vi "RemoteVI Connect VI Server.vi"(0 "window":u64, 1 "address":string) -> (4 "connected?":bool, 6 "VI":refnum<vi>, 7 "hooks":refnum<vi>, 8 "VI name":string, 9 "mode":string)   [LabVIEW 2020, in "RemoteVI.lvlib"]
doc: "The VI Server route of a window share (docs\\architecture.md, Window targets): when window belongs to ANOTHER LabVIEW process that runs VI Server, opens an application reference to it (Open Application Reference), finds the running VI whose open front panel is window - opened by the window title (a built application answers Application:All VIs In Memory with error 1032, measured), then checked with Front Panel Window:OS Window and Execution:State; a panel with a custom window title is not found and opens RemoteVI Remote Hooks.vi there from the packed library builds\\RemoteVI Hooks\\RemoteVI Hooks.lvlibp (or RemoteVI Hooks.lvlibp next to RemoteVI's folder; a built application can only load compiled code). address: empty = read the application's INI file (<exe>.ini next to the process, server.tcp.enabled=True, server.tcp.port, default 3363) and connect to 127.0.0.1; off = do not try; host:port = that VI Server. connected? TRUE: VI (the shared VI there), hooks and VI name are valid and the share runs with full features (modifier keys, tip strips, splitter bars through the hooks; everything else as for a VI of this LabVIEW). FALSE: window only; mode says why. Called by RemoteVI Server Setup.vi inside the server loop, so the references live as long as the share."
uses:
  RemoteVI.lvlib
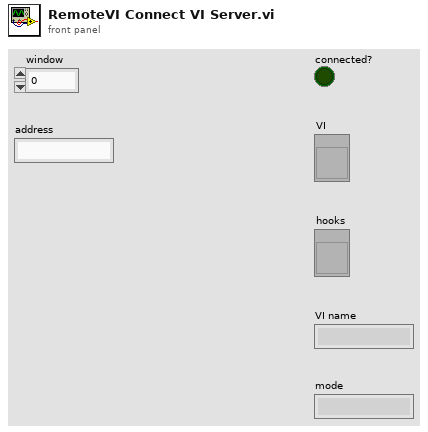
[diagram p1: front panel]
types:
  T1 = enum32{"Bad", "Idle", "Run top level", "Running"}
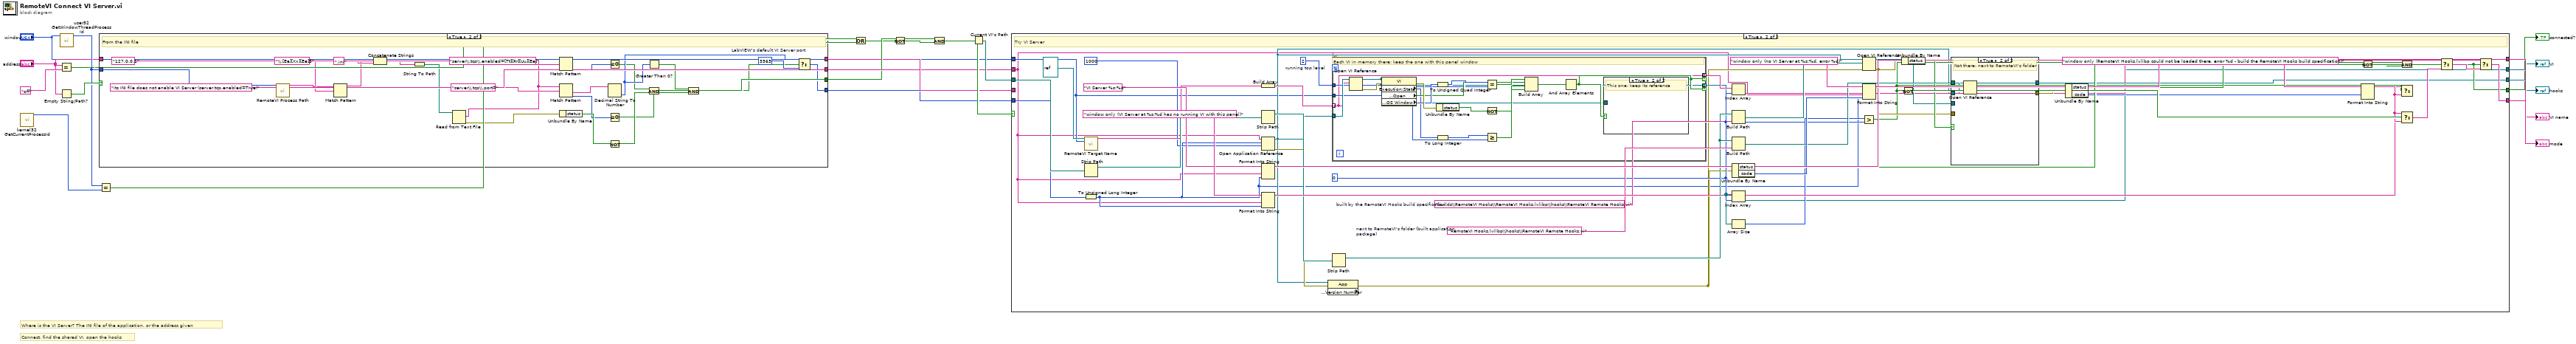
[diagram p0: block diagram]
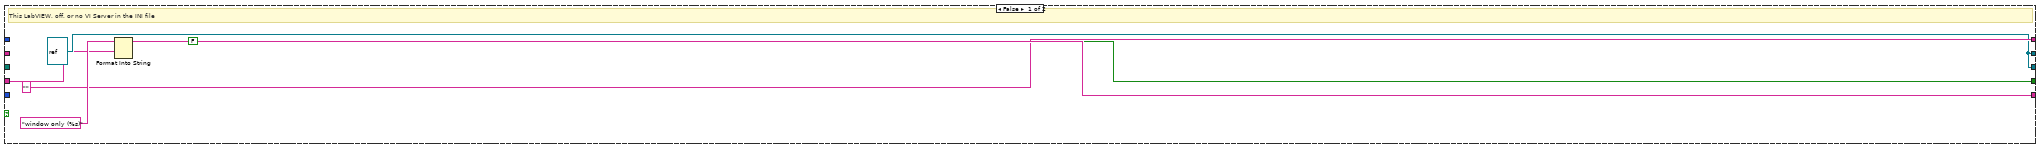
[diagram p2: hidden frame]
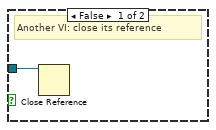
[diagram p4: hidden frame]
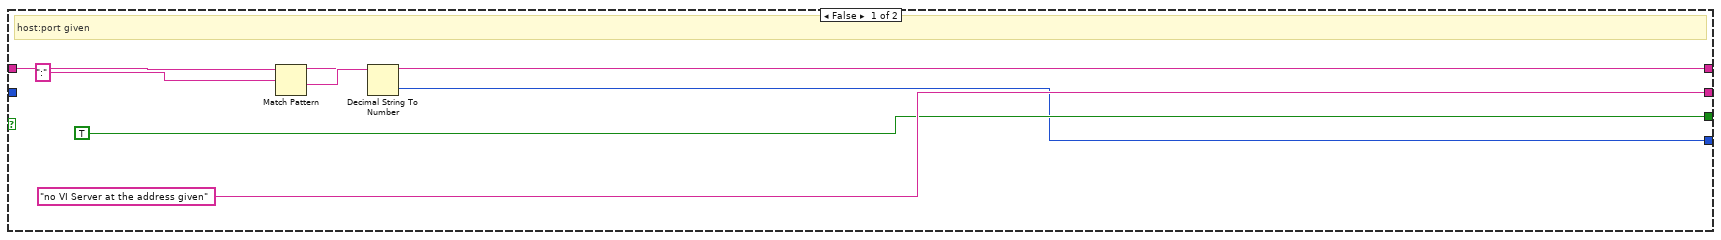
[diagram p5: hidden frame]
diagram:
  # "Connect, find the shared VI, open the hooks"
  # "Where is the VI Server? The INI file of the application, or the address given"
  n1 = call "kernel32 GetCurrentProcessId.vi"() -> ("process ID"=w4:u32)  [unwired: 14 in, 1 out]
  n2 = call "user32 GetWindowThreadProcessId.vi"("hWnd"="window") -> ("process ID"=w3:u32)  [unwired: 12 in, 2 out]
  n3 = Equal?(x="address", y="off") -> (x = y?=w7:bool)
  n4 = Empty String/Path?(string/path="address") -> (empty?=w9:bool)
  n5 = case shown="True" w9 {
    tunnel: "address" -> [w22 _]
    tunnel: [w24 "127.0.0.1"] -> w10
    tunnel: ["no VI Server at the address given" "its INI file does not enable VI Server (server.tcp.enabled=True)"] -> w13
    tunnel: w3 -> [_ w29]
    tunnel: [TRUE w52] -> w12
    tunnel: [w26 w49] -> w11
    frame False {
      # "host:port given"
      n6 = Match Pattern(string=w22, regular expression=":") -> (before substring=w24:string, after substring=w25:string)  [unwired: 1 in, 2 out]
      n7 = Decimal String To Number(string=w25) -> (number=w26:i32)  [unwired: 2 in, 1 out]
    }
    frame True {
      w48 = 3363  # LabVIEW's default VI Server port
      # "From the INI file"
      n8 = call "RemoteVI Process Path.vi"("process ID"=w29) -> ("path"=w30:string)  [unwired: 14 in]
      n9 = Match Pattern(string=w30, regular expression="\\.[Ee][Xx][Ee]$") -> (before substring=w32:string)  [unwired: 1 in, 3 out]
      n10 = Concatenate Strings(w32, ".ini") -> (w34:string)
      n11 = String To Path(string=w34) -> (path=w35:path)
      n12 = Read from Text File(file (use dialog)=w35) -> (text=w36:string, error out=w37:errorcluster)  [unwired: 3 in, 2 out]
      n13 = Match Pattern(string=w36, regular expression="server\\.tcp\\.enabled=[Tt][Rr][Uu][Ee]") -> (offset past match=w39:i32)  [unwired: 1 in, 3 out]
      n14 = Match Pattern(string=w36, regular expression="server\\.tcp\\.port=") -> (after substring=w42:string, offset past match=w43:i32)  [unwired: 1 in, 2 out]
      n15 = Unbundle By Name(w37) -> ("status"=w50:bool)
      n16 = Greater Or Equal To 0?(x=w39) -> (x >= 0?=w40:bool)
      n17 = Decimal String To Number(string=w42) -> (number=w44:i32)  [unwired: 2 in, 1 out]
      n18 = Greater Or Equal To 0?(x=w43) -> (x >= 0?=w46:bool)
      n19 = Not(x=w50) -> (.not. x?=w51:bool)
      n20 = Greater Than 0?(x=w44) -> (x > 0?=w45:bool)
      n21 = And(x=w40, y=w51) -> (x .and. y?=w52:bool)
      n22 = And(x=w45, y=w46) -> (x .and. y?=w47:bool)
      n23 = Select(t=w44, s=w47, f=w48) -> (s? t:f=w49:i32)
    }
  }
  n24 = Equal?(x=w3, y=w4) -> (x = y?=w5:bool)
  n25 = Or(x=w5, y=w7) -> (x .or. y?=w8:bool)
  n26 = Not(x=w8) -> (.not. x?=w14:bool)
  n27 = And(x=w12, y=w14) -> (x .and. y?=w15:bool)
  n28 = Current VI's Path() -> (path=w16:path)
  n29 = case shown="True" w15 {
    tunnel: "window" -> [_ w63]
    tunnel: w10 -> [_ w61]
    tunnel: w16 -> [_ w64]
    tunnel: w13 -> [w55 _]
    tunnel: ["" w78] -> w20
    tunnel: w11 -> [_ w62]
    tunnel: [w57 w77] -> w18
    tunnel: [w57 w91] -> w19
    tunnel: [FALSE w96] -> w17
    tunnel: [w60 w110] -> w21
    frame False {
      w57 = refnum<vi> refnum
      # "This LabVIEW, off, or no VI Server in the INI file"
      n30 = Format Into String(format string="window only (%s)", w55) -> (resulting string=w60:string)  [unwired: 2 in, 1 out]
    }
    frame True {
      w89 = "RemoteVI Hooks.lvlibp\\hooks\\RemoteVI Remote Hooks.vi"  # next to RemoteVI's folder (built application, package)
      w84 = "builds\\RemoteVI Hooks\\RemoteVI Hooks.lvlibp\\hooks\\RemoteVI Remote Hooks.vi"  # built by the RemoteVI Hooks build specification
      w76 = 0
      w73 = 2  # running top level
      # "Try VI Server"
      n31 = call "RemoteVI Target Name.vi"("VI"=refnum<vi> refnum, "window"=w63) -> ("name"=w71:string)  [unwired: 12 in, 1 out]
      n32 = Strip Path(path=w64) -> (stripped path=w81:path)  [unwired: 1 out]
      n33 = To Unsigned Long Integer(number=w62) -> (unsigned 32bit integer=w65:u32)
      n34 = Build Array(w71) -> (w72:string[])
      n35 = Strip Path(path=w81) -> (stripped path=w82:path)  [unwired: 1 out]
      n36 = Open Application Reference(9:1000, 10:w65, 11:w61) -> (0:w68:errorcluster, 3:w67:refnum<vi>)  [unwired: 1 in]
      n37 = Format Into String(format string="VI Server %s:%d", w61, w65) -> (resulting string=w100:string)  [unwired: 2 in, 1 out]
      n38 = Format Into String(format string="window only (VI Server at %s:%d has no running VI with this panel)", w61, w65) -> (resulting string=w104:string)  [unwired: 2 in, 1 out]
      n39 = property class="App" props=["Application:Version Number"](reference=w67, error in=w68) -> (error out=w69:errorcluster)  [unwired: 2 out]
      n40 = for {
        tunnel: w73 -> [w119]
        tunnel: w63 -> [w118]
        tunnel: w72 -> [w117] mode=indexing
        tunnel: [w117] -> w75 mode=indexing if=w134
        tunnel: w67 -> [w120]
        tunnel: [w121] -> w74 mode=indexing if=w134
        # "Each VI in memory there: keep the one with this panel window"
        n41 = Open VI Reference(application reference (local)=w120, vi path=w117) -> (vi reference=w121:refnum<vi>, error out=w122:errorcluster)  [unwired: 4 in]
        n42 = property class="VI"(reference=w121, error in=w122) -> (error out=w126:errorcluster, "Execution:State"=w123:T1, "Front Panel Window:Open"=w124:bool, "Front Panel Window:OS Window"=w125:i32)  [unwired: 1 out]
        n43 = To Unsigned Quad Integer(1:w125) -> (0:w127:u64)
        n44 = Unbundle By Name(w126) -> ("status"=w129:bool)
        n45 = To Long Integer(number=w123) -> (32bit integer=w131:i32)
        n46 = Equal?(x=w127, y=w118) -> (x = y?=w128:bool)
        n47 = Not(x=w129) -> (.not. x?=w130:bool)
        n48 = Greater Or Equal?(x=w131, y=w119) -> (x >= y?=w132:bool)
        n49 = Build Array(w128, w124, w130, w132) -> (w133:bool[])
        n50 = And Array Elements(Boolean array=w133) -> (logical AND=w134:bool)
        n51 = case shown="True" w134 {
          tunnel: w121 -> [w135 _]
          frame False {
            # "Another VI: close its reference"
            n52 = Close Reference(reference=w135) -> ()  [unwired: 1 in, 1 out]
          }
          frame True {
            # "This one: keep its reference"
          }
        }
      }
      n53 = Strip Path(path=w82) -> (stripped path=w83:path)  [unwired: 1 out]
      n54 = Index Array(array=w75, index=w76) -> (element=w78:string)
      n55 = Build Path(base path=w83, name or relative path=w84) -> (appended path=w85:path)
      n56 = Build Path(base path=w83, name or relative path=w89) -> (appended path=w90:path)
      n57 = Unbundle By Name(w69) -> ("status"=w97:bool, "code"=w98:i32)
      n58 = Index Array(array=w74, index=w76) -> (element=w77:refnum<vi>)
      n59 = Array Size(array=w74) -> (size(s)=w79:i32)
      n60 = Open VI Reference(application reference (local)=w67, vi path=w85, error in (no error)=w69) -> (vi reference=w86:refnum<vi>, error out=w87:errorcluster)  [unwired: 3 in]
      n61 = Format Into String(format string="window only (no VI Server at %s:%d, error %d)", w61, w65, w98) -> (resulting string=w102:string)  [unwired: 2 in, 1 out]
      n62 = Greater?(x=w79, y=w76) -> (0:w80:bool)
      n63 = Unbundle By Name(w87) -> ("status"=w88:bool)
      n64 = Not(x=w80) -> (.not. x?=w107:bool)
      n65 = case shown="True" w88 {
        tunnel: w90 -> [_ w114]
        tunnel: w67 -> [_ w113]
        tunnel: w86 -> [w111 _]
        tunnel: w87 -> [w112 _]
        tunnel: [w111 w115] -> w91
        tunnel: [w112 w116] -> w92
        frame False {
          # "Found in builds\\"
        }
        frame True {
          # "Not there: next to RemoteVI's folder"
          n66 = Open VI Reference(application reference (local)=w113, vi path=w114) -> (vi reference=w115:refnum<vi>, error out=w116:errorcluster)  [unwired: 4 in]
        }
      }
      n67 = Unbundle By Name(w92) -> ("status"=w93:bool, "code"=w94:i32)
      n68 = Not(x=w93) -> (.not. x?=w95:bool)
      n69 = Format Into String(format string="window only (RemoteVI Hooks.lvlibp could not be loaded there, error %d - build the RemoteVI Hooks build specification)", w94) -> (resulting string=w106:string)  [unwired: 2 in, 1 out]
      n70 = And(x=w80, y=w95) -> (x .and. y?=w96:bool)
      n71 = Select(t=w104, s=w80, f=w106) -> ()  [unwired: 1 out]
      n72 = Select(t=w104, s=w107, f=w106) -> (s? t:f=w108:string)
      n73 = Select(t=w102, s=w97, f=w108) -> (s? t:f=w109:string)
      n74 = Select(t=w100, s=w96, f=w109) -> (s? t:f=w110:string)
    }
  }
  "connected?" <- w17
  "VI" <- w18
  "hooks" <- w19
  "VI name" <- w20
  "mode" <- w21
